vi "RP1210 Send Command.vi"(7 "nMessageSize":i16, 8 "error in (no error)":errorcluster, 9 "fpchClientCommand":u8[](array[numeric])=array[4097 elements], 10 "nClientID":i16, 11 "nCommandNumber":i16) -> (0 "error out":errorcluster, 1 "fpchClientCommand out":u8[](array[numeric]), 3 "function return":i16)   [LabVIEW 2020, in "cansub_rp1210.lvlib"]
doc: "short __stdcall RP1210_SendCommand(short nCommandNumber, short nClientID, unsigned char fpchClientCommand[],\n short nMessageSize);"
uses:
  cansub_rp1210.lvlib
  cansub_lv64.dll
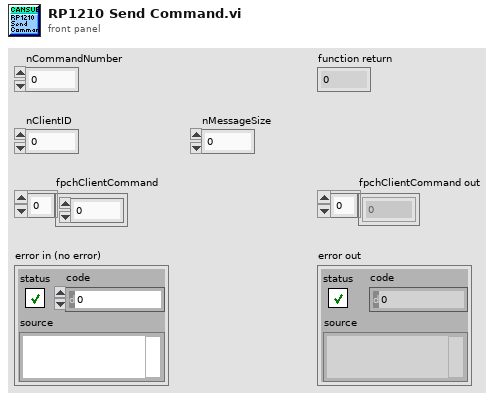
[diagram p1: front panel]
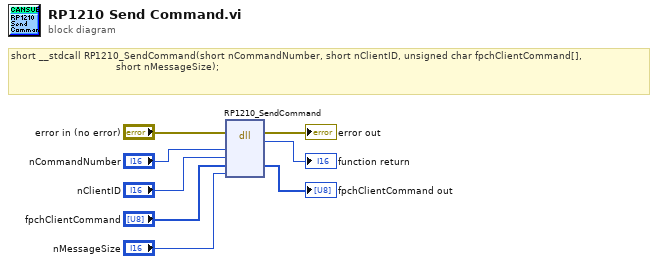
[diagram p0: block diagram]
diagram:
  # "short __stdcall RP1210_SendCommand(short nCommandNumber, short nClientID, unsigned char fpchClientCommand[],\n                                   short nMessageSize);"
  n1 = dll-call lib="C:/cansub-lv/library/cansub_lv*.*" fn="RP1210_SendCommand"(error in="error in (no error)", "nCommandNumber"="nCommandNumber", "nClientID"="nClientID", "fpchClientCommand"="fpchClientCommand", "nMessageSize"="nMessageSize") -> (error out=→"error out":errorcluster, "return type"=→"function return":i16, "fpchClientCommand"=→"fpchClientCommand out":u8[])  [unwired: 5 in, 1 out]
